vi "Make Path Relative.vi"(8 "error in":errorcluster, 10 "New Root":string, 11 "Absolute Path":path) -> (0 "error out":errorcluster, 3 "Relative Path":path)   [LabVIEW 2026]
doc: "Make path relative to the provided new root."
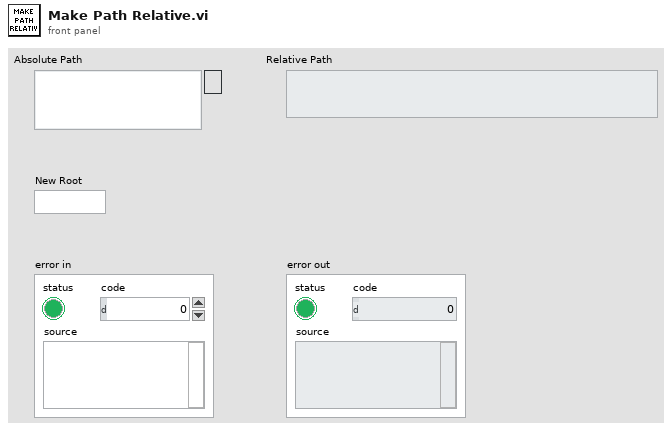
[diagram p1: front panel]
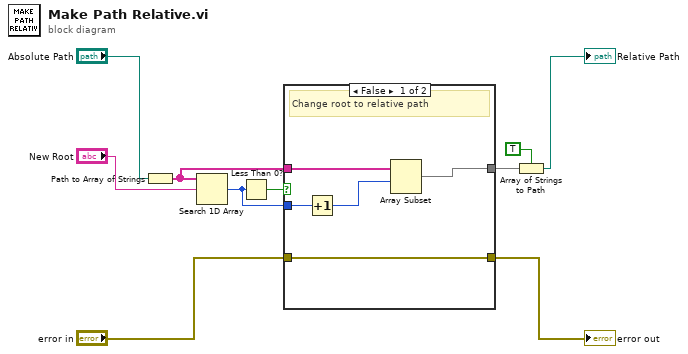
[diagram p0: block diagram]
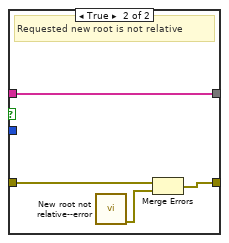
[diagram p2: hidden frame]
diagram:
  n1 = Path to Array of Strings(0:"Absolute Path") -> (2:w5:string[])  [unwired: 1 out]
  n2 = Search 1D Array(1D array=w5, element="New Root") -> (index of element=w4:i32)  [unwired: 1 in]
  n3 = Less Than 0?(x=w4) -> (x < 0?=w6:bool)
  n4 = case shown="False" w6 {
    tunnel: "error in" -> [w15 w19]
    tunnel: [w15 w17] -> w9
    tunnel: w5 -> [w14 w16]
    tunnel: w4 -> [w12 _]
    tunnel: [w13 w16] -> w3
    frame False {
      # "Change root to relative path"
      n5 = Increment(x=w12) -> (x+1=w11:i32)
      n6 = Array Subset(array=w14, index=w11) -> (w13:string[])  [unwired: 1 in]
    }
    frame True {
      # "Requested new root is not relative"
      n7 = call "New root not relative--error.vi"() -> ("error out"=w18:errorcluster)  [unwired: 11 in]
      n8 = Merge Errors(w19, w18) -> (w17:errorcluster)
    }
  }
  "error out" <- w9
  n9 = Array of Strings to Path(0:w3, 1:TRUE ("relative")) -> (2:→"Relative Path":path)
